vi "HELP Command.vi"(6 "timeout (ms) [500]":i32=500, 8 "error in (no error)":errorcluster, 10 "command":string, 11 "Instrument in":refnum<class "Instrument.lvclass">) -> (0 "error out":errorcluster, 2 "HELP out":string, 3 "Instrument in":refnum<class "Instrument.lvclass">)   [LabVIEW 2019, in "Instrument.lvlib" / "Instrument.lvclass"]
doc: "Send \"HELP\" command to get API supported by remote Instrument."
uses:
  Instrument.lvclass
  Typedefs/Instrument.Commands--Enum.ctl
  Typedefs/Instrument.HELP--Cluster.ctl
  13847043-707b-4050-995d-7bfd780093fb.vi
  13847043-707b-4050-995d-7bfd780093fb.vi/025ecd00-5096-4cec-b49a-e37656dff9da.vi
  13847043-707b-4050-995d-7bfd780093fb.vi/24fadc61-674f-4661-bc20-ce1d6faa4f48.vi
  <vilib>/Utility/Data Type/Get Type Information.vi
  <vilib>/JDP Science/JSONtext/JSON text to Variant.vi
  <vilib>/JDP Science/JSONtext/LVClass Serializer/JSONtext LVClass Serializer.lvclass
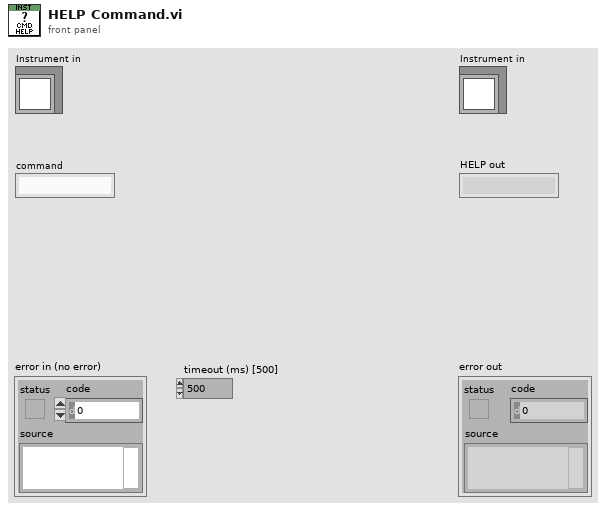
[diagram p1: front panel]
types:
  T1 = typedef "Instrument.lvlib/Instrument.lvclass/Instrument.HELP--Cluster.ctl" = cluster{"command":string}
  T2 = typedef "Instrument.lvlib/Instrument.lvclass/Instrument.Commands--Enum.ctl" = enum16{"ACK", "HELP", "IDN", "getAll", "getAllData"}
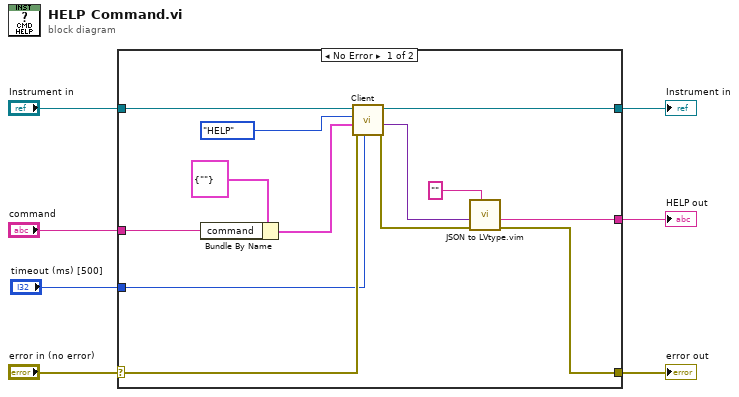
[diagram p0: block diagram]
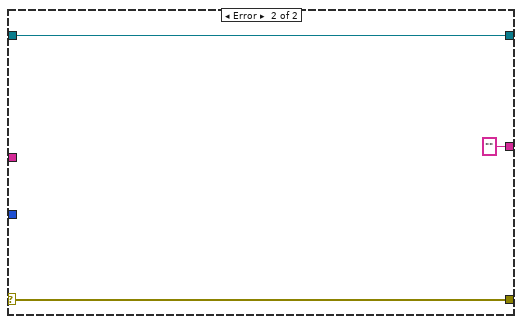
[diagram p2: hidden frame]
diagram:
  n1 = case shown="No Error" "error in (no error)" {
    selector: "error in (no error)" -> [w18 w23]
    tunnel: [w11 w23] -> w6
    tunnel: [w20 w22] -> w4
    tunnel: "Instrument in" -> [w19 w22]
    tunnel: "command" -> [w15 _]
    tunnel: [w9 "" ("Data out")] -> w2
    tunnel: "timeout (ms) [500]" -> [w8 _]
    frame No Error {
      n2 = Bundle By Name(cluster=T1 {"command"=""}, "command"=w15) -> (w14:T1)
      n3 = call-dynamic "Client.vi"("timeout (ms) [500]"=w8, "error in (no error)"=w18, "Data in"=w14, "Command in"=Instrument.Commands--Enum."HELP" ("Commands"), "Instrument in"=w19) -> ("error out"=w12:errorcluster, "Data out"=w13:variant, "Instrument out"=w20:refnum<class "Instrument.lvclass">)  [unwired: 3 in, 1 out]
      n4 = call "JSON to LVtype.vim"("type"="", "error in (no error)"=w12, "JSON Data in"=w13) -> ("error out"=w11:errorcluster, "Data out"=w9:string)  [unwired: 7 in]
    }
    frame Error {
    }
  }
  "error out" <- w6
  "Instrument in" <- w4
  "HELP out" <- w2
